vi "test_LoadCommandlineArgs_DefaultCase.vi"() -> (3 "Pass?":bool)   [LabVIEW 2019, in "Tests.SolutionBuilder.lvlib"]
uses:
  Tests.SolutionBuilder.lvlib
  SolutionBuilder/Community/Options.ctl
  SolutionBuilder/SolutionBuilder.lvclass
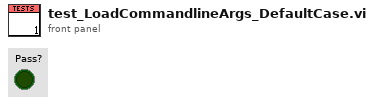
[diagram p1: front panel]
types:
  T1 = typedef "SolutionBuilder.lvlib/SolutionBuilder.lvclass/Options.ctl" = cluster{"Path":path, "Preview?":bool, "Quiet?":bool, "Log file":path, "Success file":path, "Rebuild?":bool, "Keep split projects?":bool}
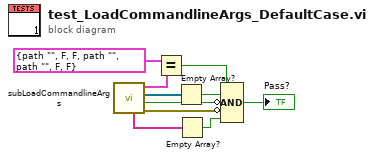
[diagram p0: block diagram]
diagram:
  n1 = call "subLoadCommandlineArgs.vi"() -> ("error out"=w10:errorcluster, "From command line?"=w8:bool, "Pre-built libraries"=w5:refnum<class "ProjectItem.lvclass">[], "Options"=w3:T1, "Active targets"=w2:string[])  [unwired: 7 in]
  n2 = Equal?(x=T1 {"Path"=path "", "Preview?"=FALSE, "Quiet?"=FALSE, "Log file"=path "", "Success file"=path "", "Rebuild?"=FALSE, "Keep split projects?"=FALSE} ("Options"), y=w3) -> (x = y?=w7:bool)
  n3 = Empty Array?(array=w5) -> (empty?=w6:bool)
  n4 = Empty Array?(array=w2) -> (empty?=w1:bool)
  n5 = Compound Arithmetic op=AND(w7, w6, invert w8, invert w10, w1) -> (→"Pass?":bool)
